vi "Handle Update App.vi"(7 "Sort Order":T1, 8 "error in (no error)":errorcluster, 10 "ViaApp":refnum<class "ViaApp.lvclass">, 11 "AppListPanel in":refnum<class "AppListPanel.lvclass">) -> (0 "error out":errorcluster, 3 "AppListPanel out":refnum<class "AppListPanel.lvclass">)   [LabVIEW 2020, in "PicoG-App.lvlib" / "AppListPanel.lvclass"]
uses:
  AppListPanel.lvclass
  ViaApp/ViaApp.lvclass
  Sort Order.ctl
  AppListPanel.lvclass/AppListPanel.ctl
  GWebAppArrayPanel/GWebAppArrayPanel.lvclass
  C:/Program Files (x86)/National Instruments/LabVIEW 2020/vi.lib/IlluminatedG/IG OOPanel/OOPanel/ArrayPanel/ArrayPanel.lvclass
  App Panel.ctl
  <vilib>/IlluminatedG/IG OOPanel/OOPanel/ArrayManager/ArrayManager.lvclass
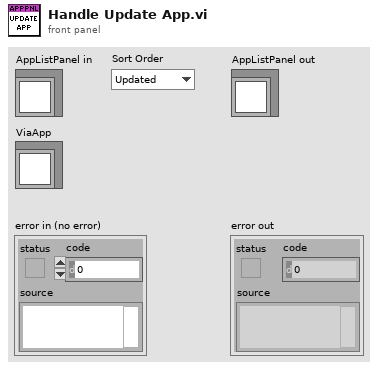
[diagram p1: front panel]
types:
  T1 = typedef "PicoG-App.lvlib/AppListPanel.lvclass/Sort Order.ctl" = enum16{"Updated", "Name"}
  T2 = typedef "PicoG-App.lvlib/AppListPanel.lvclass/App Panel.ctl" = cluster{"App":refnum<class "ViaApp.lvclass">, "Panel":refnum<class "GWebAppArrayPanel.lvclass">}
  T3 = typedef "PicoG-App.lvlib/AppListPanel.lvclass/Ref Data.ctl" = cluster{"App Map":map{path, T2}}
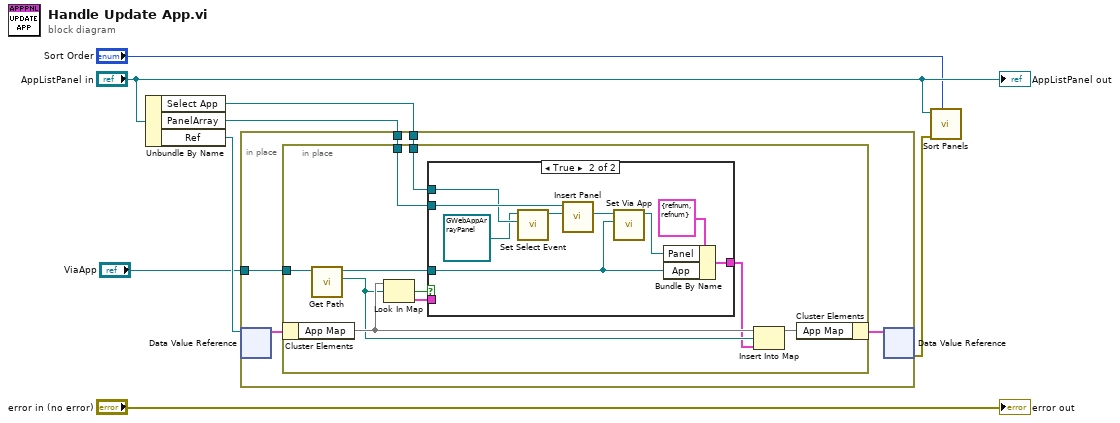
[diagram p0: block diagram]
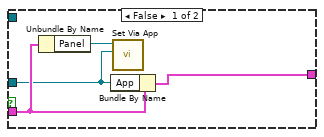
[diagram p2: hidden frame]
diagram:
  n1 = Unbundle By Name("AppListPanel in") -> ("Select App"=w2:refnum<user-event>, "PanelArray"=w3:refnum<class "ArrayManager.lvclass">, "Ref"=w7:refnum<data-value>)
  n2 = in-place {
    in-place-border: "ViaApp" -> [w11]
    in-place-border: w3 -> [w10]
    in-place-border: w2 -> [w9]
    n3 = in-place-dvr #1(w7) -> (w13:T3)  [unwired: 1 out]
    n4 = in-place {
      in-place-border: w11 -> [w23]
      in-place-border: w10 -> [w20]
      in-place-border: w9 -> [w18]
      n5 = in-place-cluster #2(w13) -> ("App Map"=w17:map{path, T2})
      n6 = call "Get Path.vi"("ViaApp in"=w23) -> ("Path"=w16:path, "ViaApp out"=w22:refnum<class "ViaApp.lvclass">)  [unwired: 8 in, 1 out]
      n7 = Look In Map(map=w17, key=w16) -> (key not found?=w21:bool, value=w19:T2)  [unwired: 1 in]
      n8 = case shown="True" w21 {
        tunnel: w22 -> [w24 w32]
        tunnel: w20 -> [_ w35]
        tunnel: w19 -> [w26 _]
        tunnel: w18 -> [_ w33]
        tunnel: [w27 w31] -> w15
        frame False {
          n9 = Unbundle By Name(w26) -> ("Panel"=w25:refnum<class "GWebAppArrayPanel.lvclass">)
          n10 = Bundle By Name(cluster=w26, "App"=w24) -> (w27:T2)
          n11 = call "Set Via App.vi"("ViaApp"=w24, "GWebAppArrayPanel in"=w25) -> ()  [unwired: 8 in, 2 out]
        }
        frame True {
          n12 = call "Set Select Event.vi"("Select App Event"=w33, "GWebAppArrayPanel in"=refnum<class "GWebAppArrayPanel.lvclass"> refnum ("PicoG-App.lvlib:GWebAppArrayPanel.lvclass")) -> ("GWebAppArrayPanel out"=w29:refnum<class "GWebAppArrayPanel.lvclass">)  [unwired: 8 in, 1 out]
          n13 = call <vilib>:"Insert Panel.vi"("Panel/Type"=w29, "PanelArray in"=w35) -> ("Panel"=w36:refnum<class "GWebAppArrayPanel.lvclass">)  [unwired: 7 in, 2 out]
          n14 = call "Set Via App.vi"("ViaApp"=w32, "GWebAppArrayPanel in"=w36) -> ("GWebAppArrayPanel out"=w28:refnum<class "GWebAppArrayPanel.lvclass">)  [unwired: 8 in, 1 out]
          n15 = Bundle By Name(cluster=T2 {"App"=refnum, "Panel"=refnum} ("App Panel"), "Panel"=w28, "App"=w32) -> (w31:T2)
        }
      }
      n16 = Insert Into Map(map in=w17, key=w16, value=w15) -> (map out=w14:map{path, T2})  [unwired: 2 out]
      n17 = in-place-cluster #2("App Map"=w14) -> (w12:T3)
    }
    n18 = in-place-dvr #1(w12) -> (w1:errorcluster)  [unwired: 1 out]
  }
  n19 = call "Sort Panels.vi"("Sort Order"="Sort Order", "error in (no error)"=w1, "AppListPanel"="AppListPanel in") -> ()  [unwired: 8 in, 1 out]
  "error out" <- "error in (no error)"
  "AppListPanel out" <- "AppListPanel in"
